vi "Embedded Webview.vi"() -> ()   [LabVIEW 2026]
doc: "Uses a Web Browser to display web content."
panel:
  in  "To Web Page":u16
  out "URL":string="http://localhost:5173/"
  out "Exception":string
  out "Web Browser Control":string(html)="http://localhost:5173/"
  out "From Web Page":u16
  in  "Stop":bool
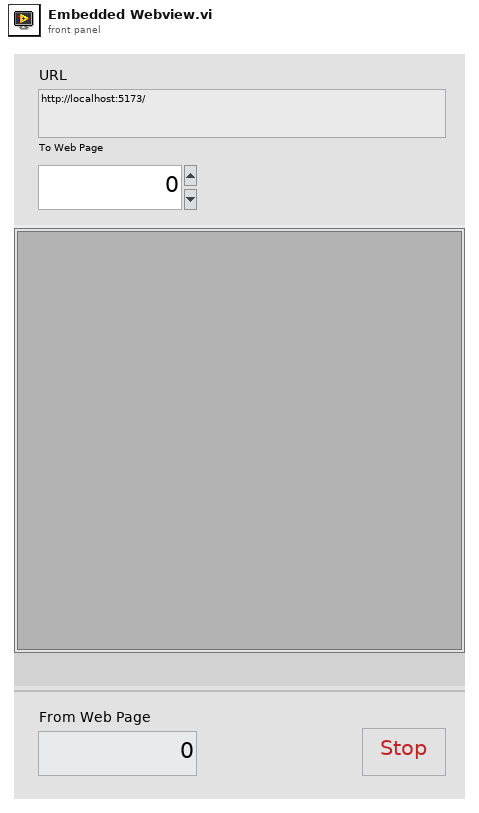
[diagram p1: front panel]
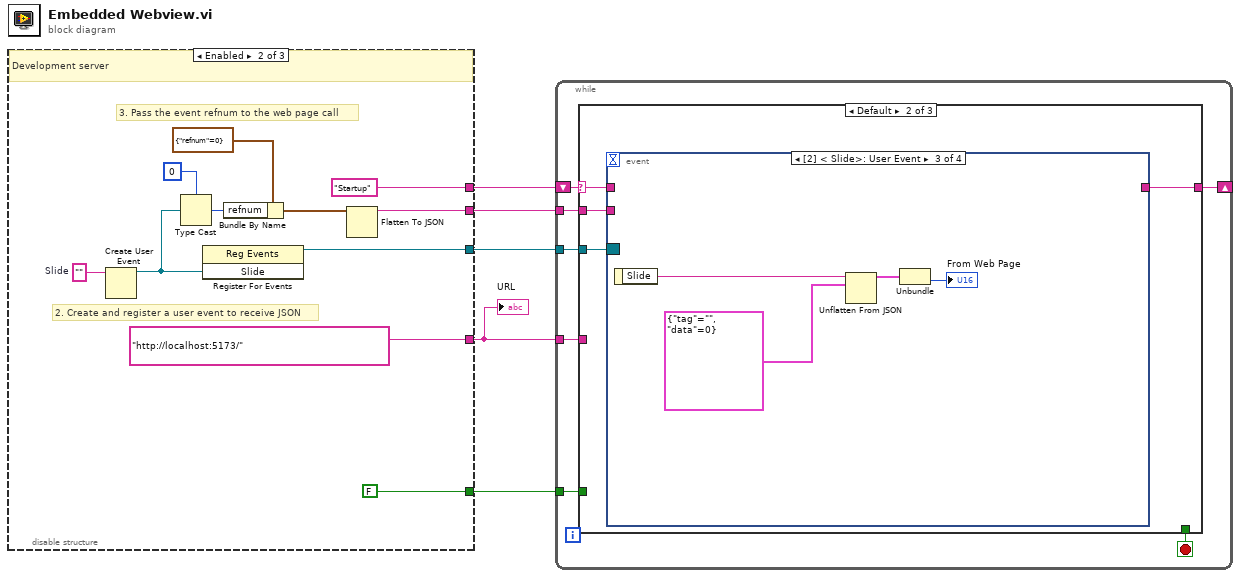
[diagram p0: block diagram]
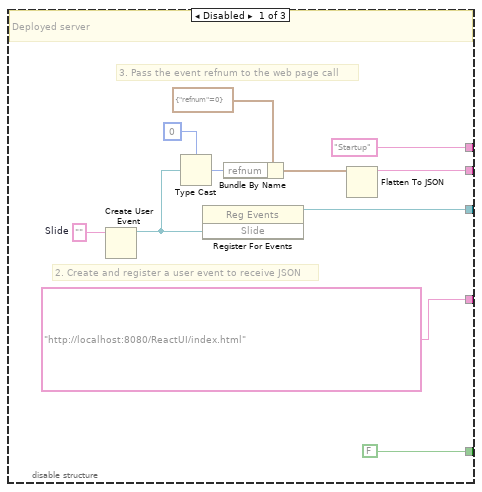
[diagram p2: hidden frame]
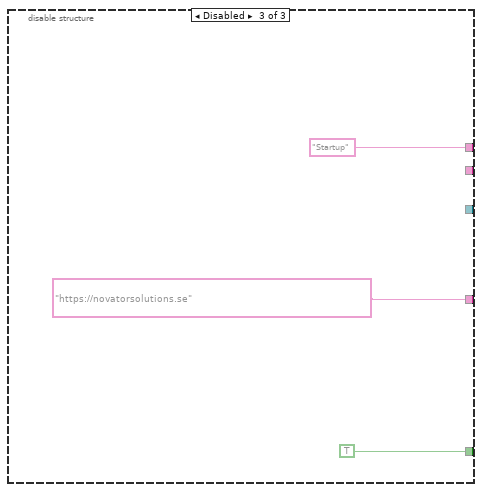
[diagram p3: hidden frame]
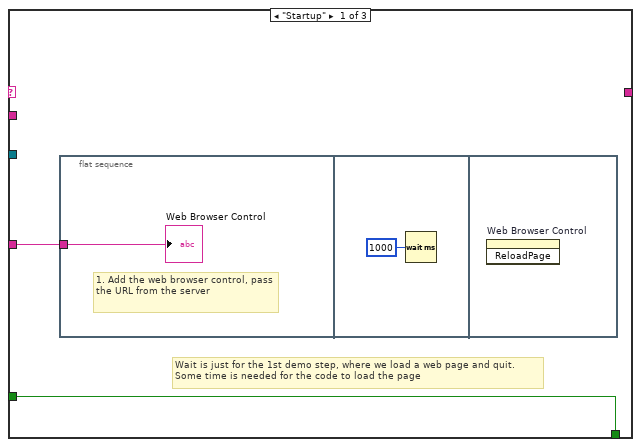
[diagram p4: hidden frame]
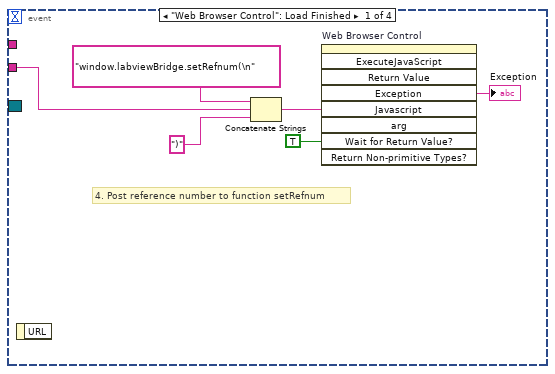
[diagram p5: hidden frame]
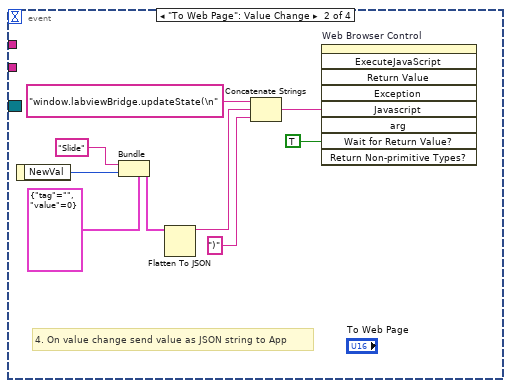
[diagram p6: hidden frame]
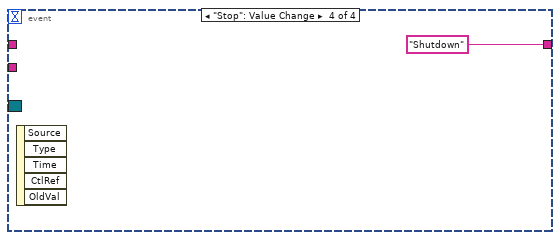
[diagram p7: hidden frame]
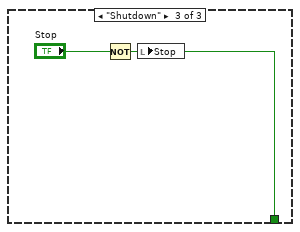
[diagram p8: hidden frame]
diagram:
  n1 = disable-structure shown="Enabled" {
    disable-tunnel: ["Startup" "Startup" "Startup"] -> w5
    disable-tunnel: [w14 w25 _] -> w4
    disable-tunnel: [w9 w20 _] -> w3
    disable-tunnel: [FALSE ("Stop 2") FALSE ("Stop 2") TRUE ("Stop 2")] -> w2
    disable-tunnel: ["http://localhost:8080/ReactUI/index.html" ("URL") "http://localhost:5173/" ("URL") "https://novatorsolutions.se" ("URL")] -> w1
    frame Disabled {
      w16 = ""  # Slide
      # "3. Pass the event refnum to the web page call"
      # "2. Create and register a user event to receive JSON"
      # "Deployed server"
      n2 = Create User Event(user event datatype=w16) -> (user event=w8:refnum<user-event>)  [unwired: 1 in, 1 out]
      n3 = Type Cast(type=u32 0, x=w8) -> (*(type *) &x=w10:u32)
      n4 = register-events(w8) -> (reference out=w14:refnum<event-registration>)  [unwired: 2 in, 1 out]
      n5 = Bundle By Name(cluster=cluster{"refnum":u32} {"refnum"=0}, "refnum"=w10) -> (w12:cluster{"refnum":u32})
      n6 = Flatten To JSON(anything=w12) -> (JSON string=w9:string)  [unwired: 2 in, 1 out]
    }
    frame Enabled {
      w27 = ""  # Slide
      # "3. Pass the event refnum to the web page call"
      # "2. Create and register a user event to receive JSON"
      # "Development server"
      n7 = Create User Event(user event datatype=w27) -> (user event=w19:refnum<user-event>)  [unwired: 1 in, 1 out]
      n8 = Type Cast(type=u32 0, x=w19) -> (*(type *) &x=w21:u32)
      n9 = register-events(w19) -> (reference out=w25:refnum<event-registration>)  [unwired: 2 in, 1 out]
      n10 = Bundle By Name(cluster=cluster{"refnum":u32} {"refnum"=0}, "refnum"=w21) -> (w23:cluster{"refnum":u32})
      n11 = Flatten To JSON(anything=w23) -> (JSON string=w20:string)  [unwired: 2 in, 1 out]
    }
    frame Disabled {
    }
  }
  "URL" <- w1
  n12 = while {
    shift-right: [w36] -> _
    shift-left: w5 -> [w37]
    tunnel: w4 -> [w35]
    tunnel: w3 -> [w34]
    tunnel: w2 -> [w32]
    tunnel: w1 -> [w31]
    stop <- w33 stop-if-true
    n13 = case shown="Default" w37 {
      selector: w37 -> [_ w45 _]
      tunnel: [_ w44 _] -> w36
      tunnel: w35 -> [_ w43 _]
      tunnel: w34 -> [_ w42 _]
      tunnel: [w39 _ "Stop"] -> w33
      tunnel: w32 -> [w39 _ _]
      tunnel: w31 -> [w38 _ _]
      frame "Startup" {
        # "Wait is just for the 1st demo step, where we load a web page and quit.\nSome time is needed for the code to load the page"
        n14 = flat-sequence {
          tunnel: w38 -> [w40]
          frame #0 {
            # "1. Add the web browser control, pass the URL from the server"
            "Web Browser Control" <- w40
          }
          frame #1 {
            n15 = Wait (ms)(milliseconds to wait=u32 1000) -> ()  [unwired: 1 out]
          }
          frame #2 {
            n16 = invoke on="Web Browser Control" class="WebBrowser (strict)" method="ReloadPage"() -> ()  [unwired: 3 in, 3 out]
          }
        }
      }
      frame Default {
        n17 = event shown="[2] < Slide>: User Event" {
          selector: w43 -> [_ _ _ _]
          dyn-events: _ -> [_ _ _ _]
          timeout: _ -> [_ _ _ _]
          tunnel: w45 -> [_ _ _ _]
          tunnel: [_ _ _ "Shutdown"] -> w44
          tunnel: w42 -> [w49 _ _ _]
          event "Web Browser Control": Load Finished {
            # "4. Post reference number to function setRefnum"
            n18 = event-data() -> ()  [unwired: 1 in, 1 out]
            n19 = Concatenate Strings("window.labviewBridge.setRefnum(\n" ("Javascript String"), w49, ")" ("string")) -> (w47:string)
            n20 = invoke on="Web Browser Control" class="WebBrowser (strict)" method="ExecuteJavaScript"("Javascript"=w47, "Wait for Return Value?"=TRUE) -> ("Exception"=→"Exception":string)  [unwired: 7 in, 8 out]
          }
          event "To Web Page": Value Change {
            # "4. On value change send value as JSON string to App"
            n21 = event-data() -> ("NewVal"=w53:u16)  [unwired: 1 in]
            n22 = Bundle(cluster=cluster{"tag":string, "value":u16} {"tag"="", "value"=0}, "tag"="Slide", "value"=w53) -> (w54:cluster{"tag":string, "value":u16})
            n23 = Flatten To JSON(anything=w54) -> (JSON string=w55:string)  [unwired: 2 in, 1 out]
            n24 = Concatenate Strings("window.labviewBridge.updateState(\n" ("Javascript String"), w55, ")" ("string")) -> (w57:string)
            n25 = invoke on="Web Browser Control" class="WebBrowser (strict)" method="ExecuteJavaScript"("Javascript"=w57, "Wait for Return Value?"=TRUE) -> ()  [unwired: 7 in, 9 out]
          }
          event User Event {
            n26 = event-data() -> ("Slide"=w64:string)  [unwired: 1 in]
            n27 = Unflatten From JSON(JSON string=w64, type and defaults=cluster{"tag":string, "data":u16} {"tag"="", "data"=0}) -> (value=w62:cluster{"tag":string, "data":u16})  [unwired: 5 in, 1 out]
            n28 = Unbundle(w62) -> ("data"=→"From Web Page":u16)  [unwired: 1 out]
          }
          event "Stop": Value Change {
            n29 = event-data() -> ()  [unwired: 1 in, 5 out]
          }
        }
      }
      frame "Shutdown" {
        n30 = Not(x="Stop") -> (.not. x?=w66:bool)
        n31 = local write "Stop"(w66) -> ()
      }
    }
  }
